vi "UI (Experienced).vi"() -> ()   [LabVIEW 2017, in "UI.lvlib"]
doc: "The Queued Message Handler of a Worker."
uses:
  UI.lvlib
  _support/Analysis Window Type.ctl
  _support/UI State.ctl
  1af51285-6659-428e-9c15-de70f1a207c9.vi
  1756710f-d813-4077-a3f9-6f06171a4225.vi
  b1498353-a107-4479-98d0-7e76c0451ff6.vi
  242d01f8-d211-4c25-bb6c-8191a2acbe42.vi
  da0d510b-1f54-4e49-9d1f-893e7e8abfcf.vi
  e403ca69-710b-4b23-8527-f02bfa86df9b.vi
  <userlib>/_NEVSTOP/Communicable State Machine(CSM)/AdvanceAPI/CSM - Revert Arguments-Safe String.vi
  <userlib>/_NEVSTOP/Communicable State Machine(CSM)/_Shared/Trim Single-line Text.vi
  <userlib>/_NEVSTOP/Communicable State Machine(CSM)/AdvanceAPI/CSM - Make String Arguments Safe.vi
  <userlib>/_NEVSTOP/Communicable State Machine(CSM)/AdvanceAPI/CSM - Break Down Multiple States String.vi
  <userlib>/_NEVSTOP/Communicable State Machine(CSM)/AdvanceAPI/CSM - Keywords.vi
  <userlib>/_NEVSTOP/Communicable State Machine(CSM)/addons/INI-Static-Variable-Support/_Support/instances/_CSM - Read File Logger Configuration - v1.0.vi
  <userlib>/_NEVSTOP/Communicable State Machine(CSM)/addons/API-String-Arugments-Support/_Support/Convert API String Arguments to Data(variant).vi
  <userlib>/_NEVSTOP/Communicable State Machine(CSM)/addons/API-String-Arugments-Support/_Support/Query Data as API String Arguments(variant).vi
  <userlib>/_NEVSTOP/Communicable State Machine(CSM)/addons/MassData-Parameter/_support/FGV-MassData(lvlibp).vi
  <userlib>/_NEVSTOP/Communicable State Machine(CSM)/_Polymophic/Add State(s) to Queue By BOOL(Element).vi
  <userlib>/_NEVSTOP/Communicable State Machine(CSM)/_Polymophic/CSM - Replace Marks in Messages.vi
  Acquisition/Acquisition.lvlib
  Logging/Logging.lvlib
  <userlib>/_NEVSTOP/Communicable State Machine(CSM)/Communicable State Machine.lvlib
  <userlib>/_NEVSTOP/Communicable State Machine(CSM)/addons/MassData-Parameter/CSM MassData Parameter Support.lvlib
  <userlib>/_NEVSTOP/Communicable State Machine(CSM)/addons/INI-Static-Variable-Support/INI-Static-Variable-Support.lvlib
  Algorithm/Algorithm.lvlib
  <userlib>/_NEVSTOP/Communicable State Machine(CSM)/addons/Logger/CSM File Logger.lvlib
  <userlib>/_NEVSTOP/Communicable State Machine(CSM)/addons/Watchdog/CSM Watchdog.lvlib
  <userlib>/_NEVSTOP/Communicable State Machine(CSM)/_Polymophic/Build Synchronous Message with Arguments.vi
panel:
  out "WaveformGraph":waveform(dbl)[](graph)
  in  "Analysis Window 1":T1
  out "AnalysisWnd 1":cluster{"f0":dbl, "df":dbl, "magnitude":dbl[]}[](graph)
  in  "Analysis Window 2":T1
  out "AnalysisWnd 2":cluster{"f0":dbl, "df":dbl, "magnitude":dbl[]}[](graph)
  in  "Settings":bool
  in  "Start":bool
  in  "Stop":bool
  out "Status":string
  in  "Exit":bool
  # "Continuous Measurement and Data Logger - CSM Version"
  # "Experienced Example"
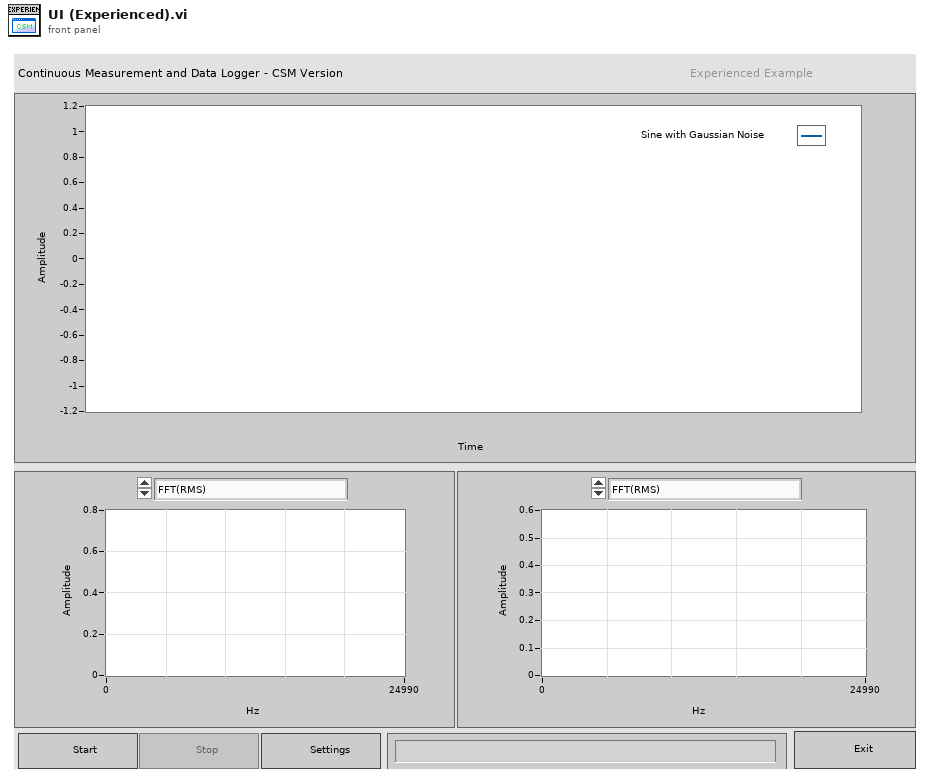
[diagram p1: front panel]
types:
  T1 = typedef "UI.lvlib/Analysis Window Type.ctl" = enum16{"FFT(RMS)", "FFT(Peak)", "Power Spectrum"}
  T2 = cluster{"Enable":bool, "Limit":cluster{"FileSize":i64, "FileNum":i32}, "Timestamp.Format":string, "AutoExit":bool}
  T3 = enum32{"Invalid", "Standard", "Closed", "Hidden", "Minimized", "Maximized"}
  T4 = enum32{"invalid app kind", "Development System", "Run Time System", "Student Edition", "Embedded LabVIEW", "Evaluation", "Custom"}
  T5 = typedef "UI.lvlib/UI State.ctl" = enum16{"Idle", "Acquiring and Logging", "Waiting for Exit", "Waiting for Exit (Acq Stopped)", "Waiting for Exit (Log Stopped)", "Waiting for Stop", "Waiting for Stop (Acq Stopped)", "Waiting for Stop (Log Stopped)"}
  T6 = enum32{"Invalid", "Default", "Floating", "Floating/Auto-Hide", "Modal"}
  T7 = typedef "Communicable State Machine.lvlib/_CSM_Response Source Message.ctl" = cluster{"‘State":string, "’Arguments":string, "’Error":errorcluster}
  T8 = cluster{"Current VI Reference":refnum<vi>, "Close Panel on Exit?":bool}
  T9 = cluster{"Core":cluster{"Current VI Reference":refnum<vi>, "Close Panel on Exit?":bool}, "UI Refs":cluster{"Start Ref":refnum<vi>, "Stop Ref":refnum<vi>, "Settings Ref":refnum<vi>, "Exit Ref":refnum<vi>, "Status Ref":refnum<vi>, "Data Ref":refnum<vi>, "Data Source Ref":refnum<vi>}, "State":T5, "Relationships":string}
  T10 = cluster{"Start Ref":refnum<vi>, "Stop Ref":refnum<vi>, "Settings Ref":refnum<vi>, "Exit Ref":refnum<vi>, "Status Ref":refnum<vi>, "Data Ref":refnum<vi>, "Data Source Ref":refnum<vi>}
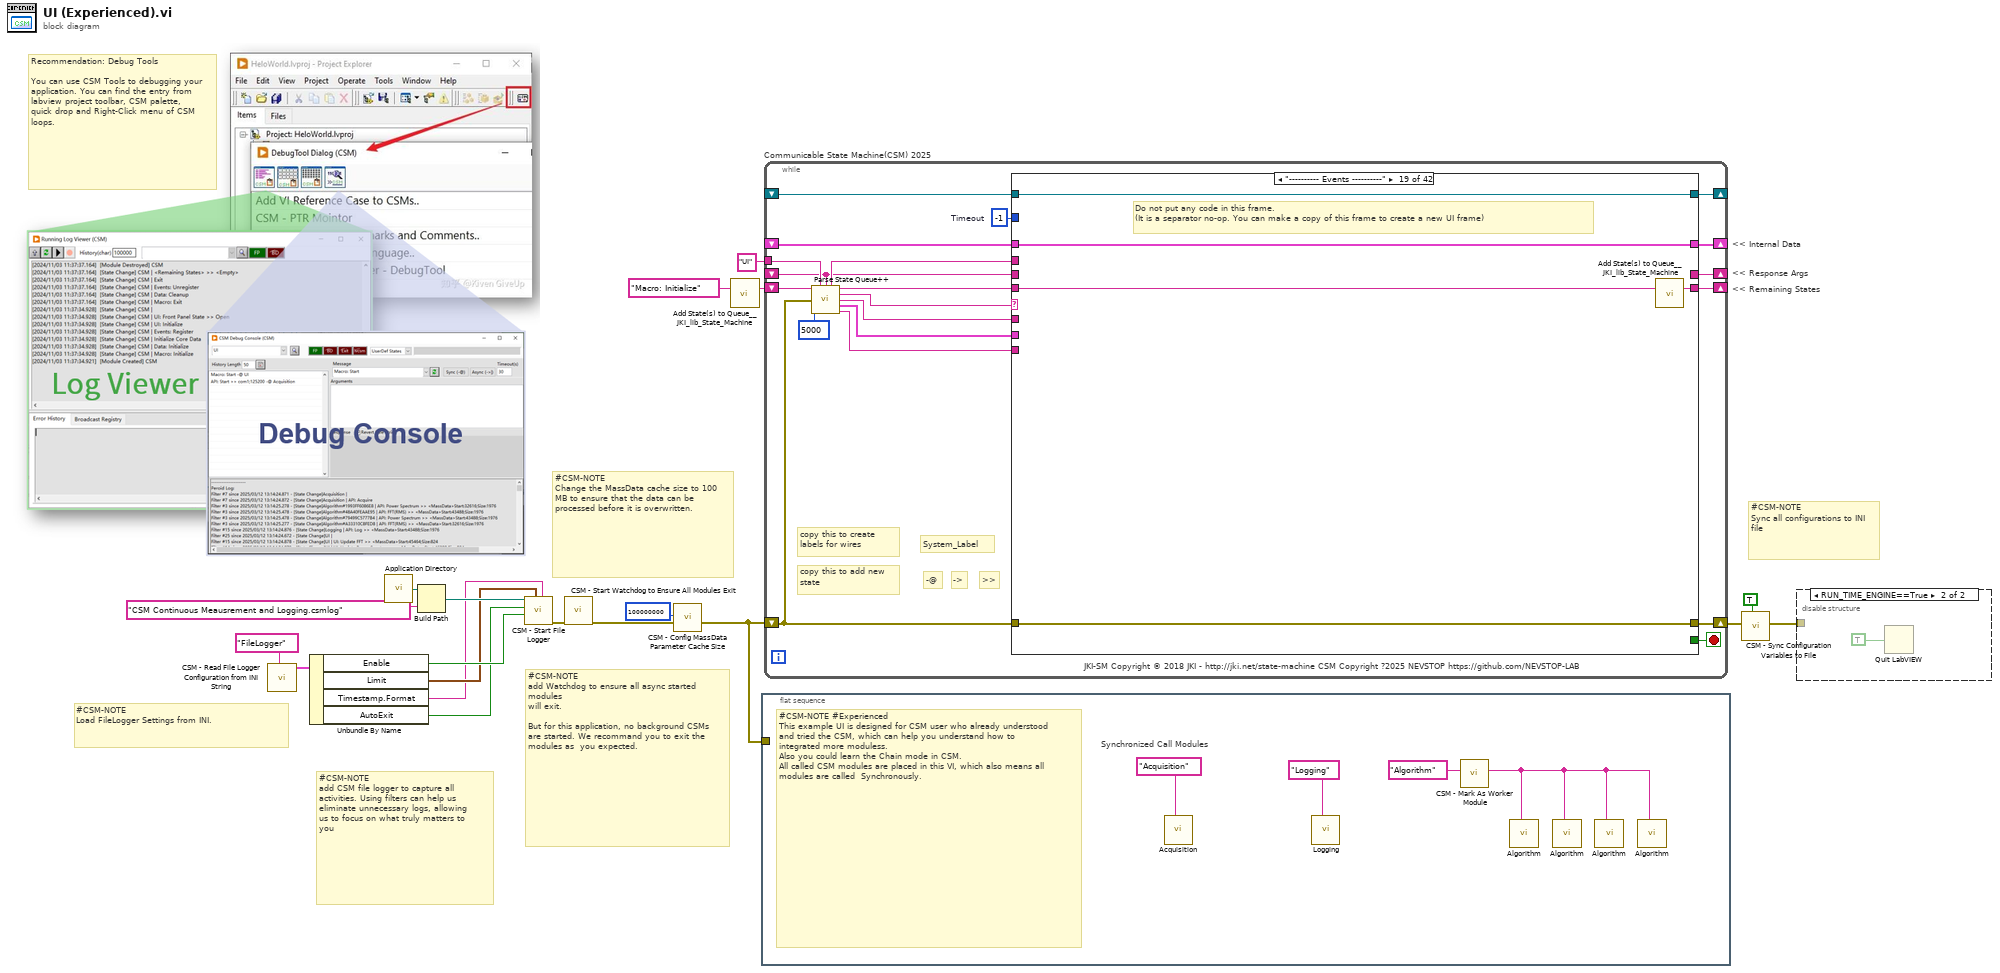
[diagram p0: block diagram]
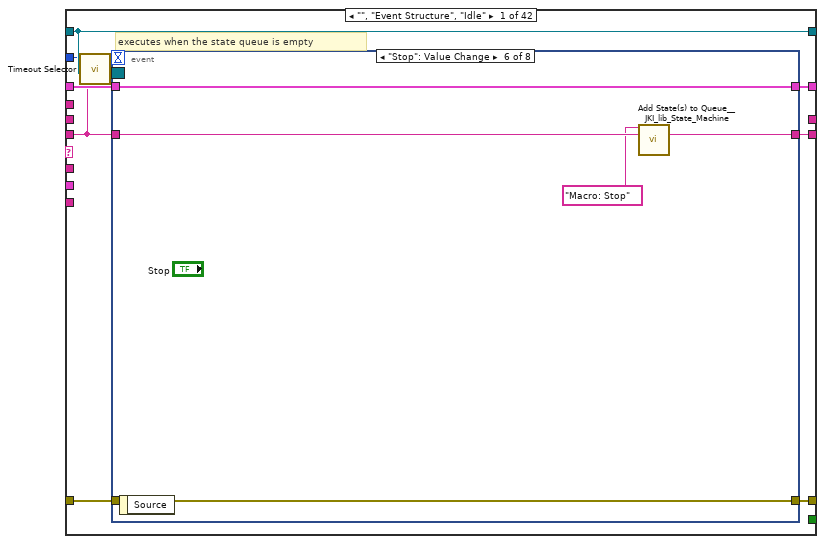
[diagram p3: hidden frame]
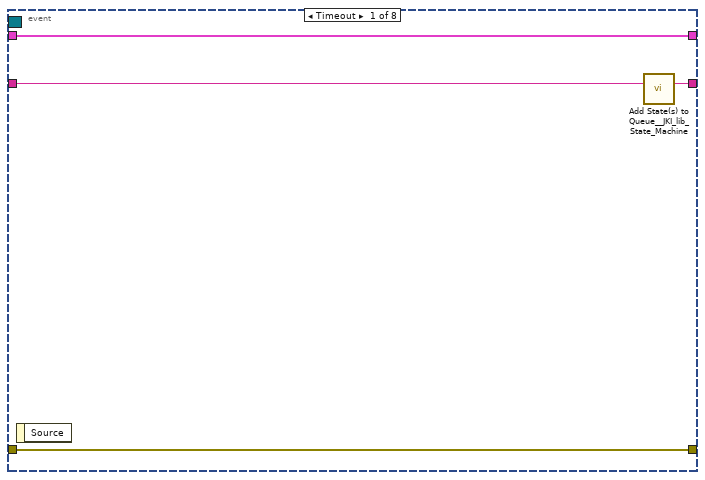
[diagram p4: hidden frame]
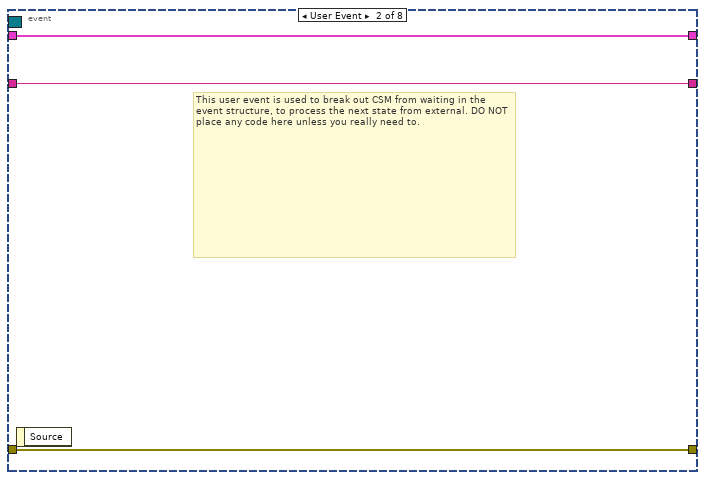
[diagram p5: hidden frame]
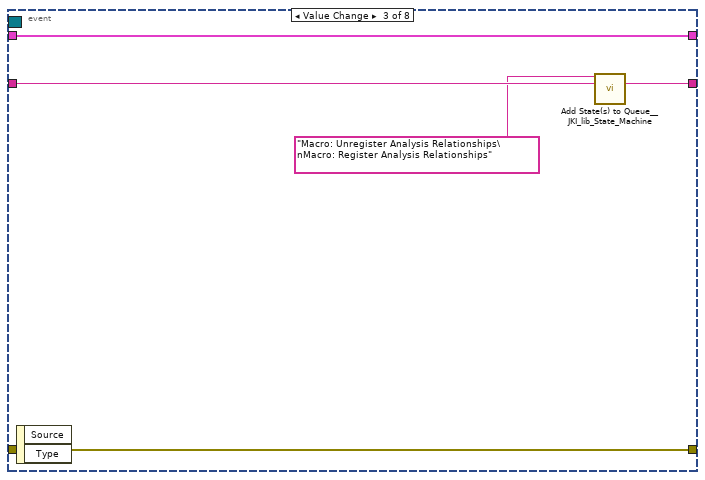
[diagram p6: hidden frame]
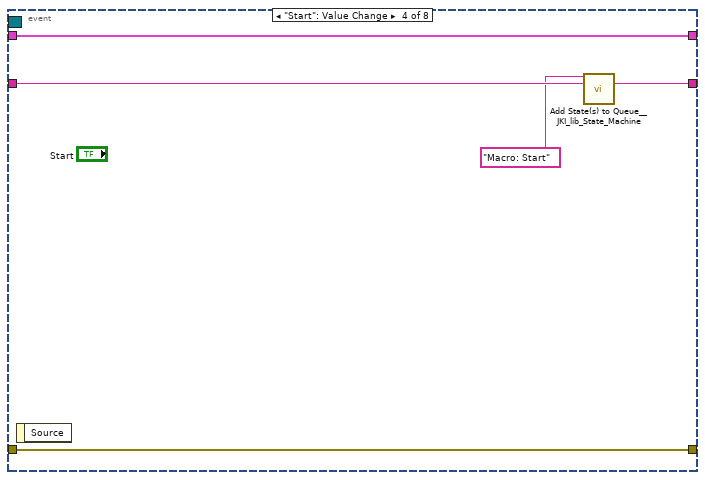
[diagram p7: hidden frame]
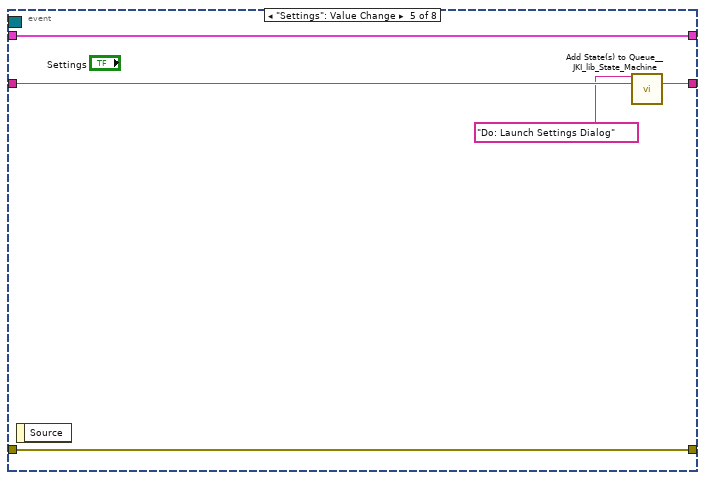
[diagram p8: hidden frame]
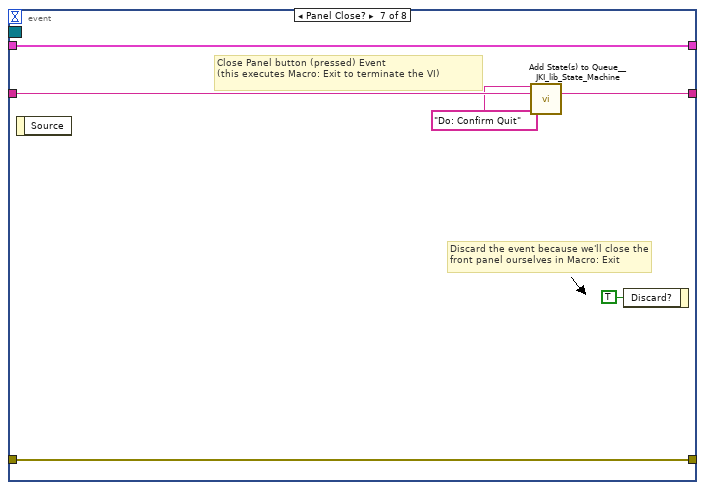
[diagram p9: hidden frame]
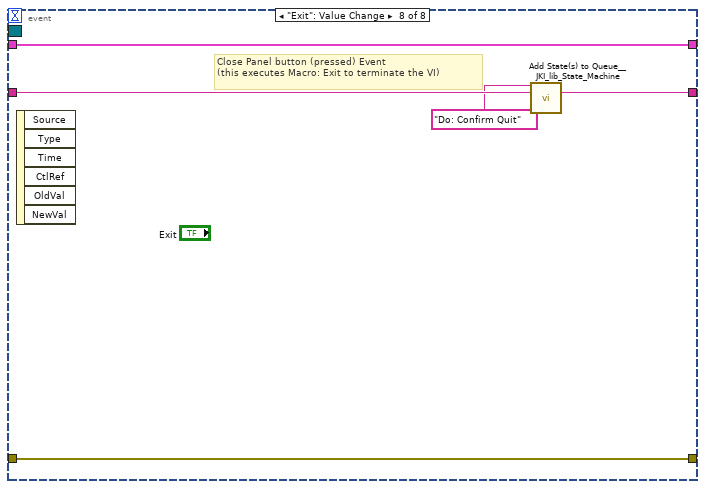
[diagram p10: hidden frame]
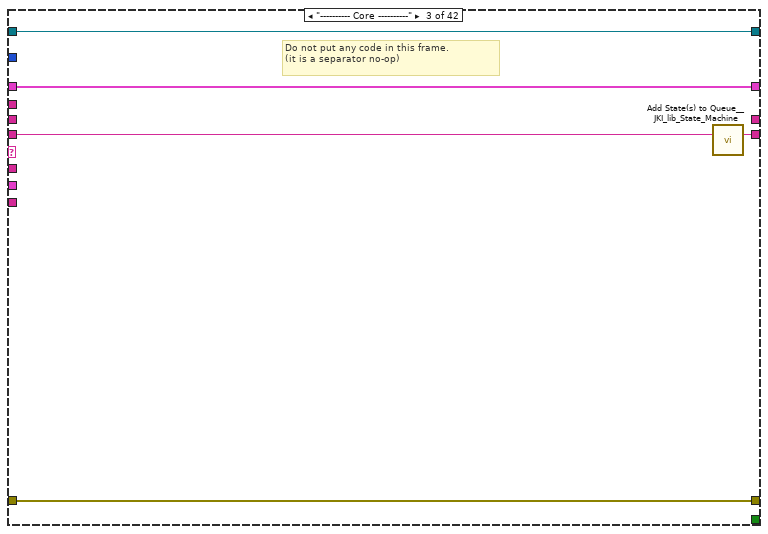
[diagram p12: hidden frame]
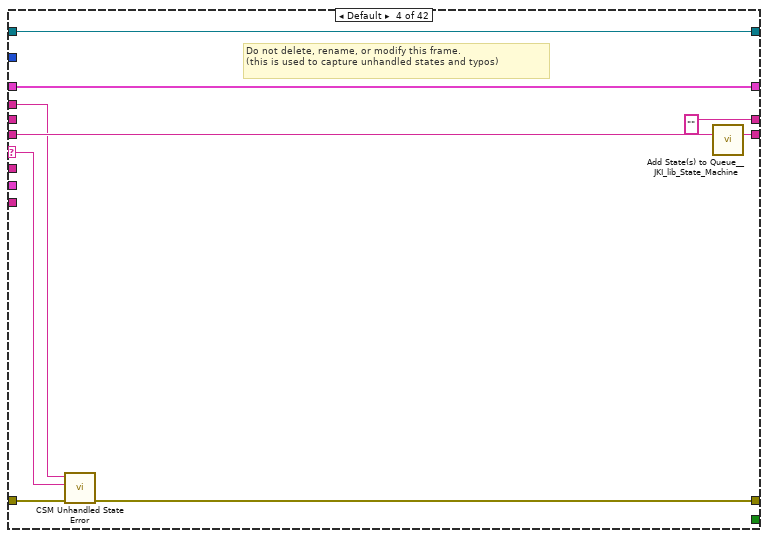
[diagram p13: hidden frame]
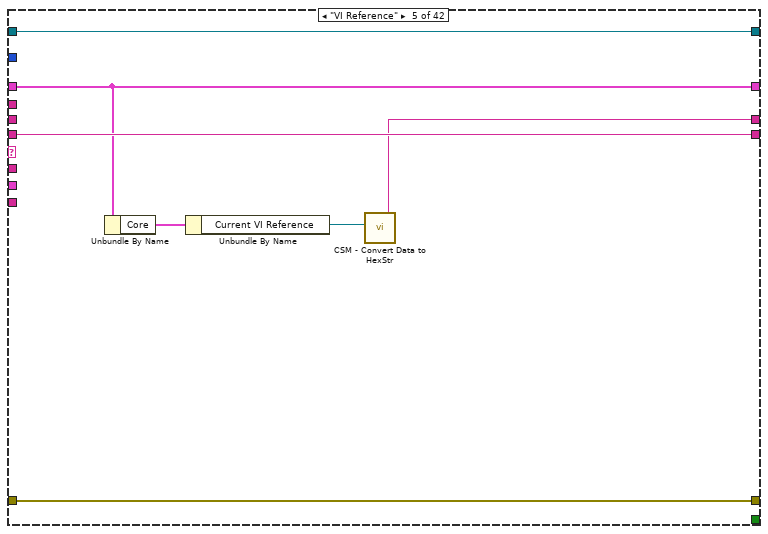
[diagram p14: hidden frame]
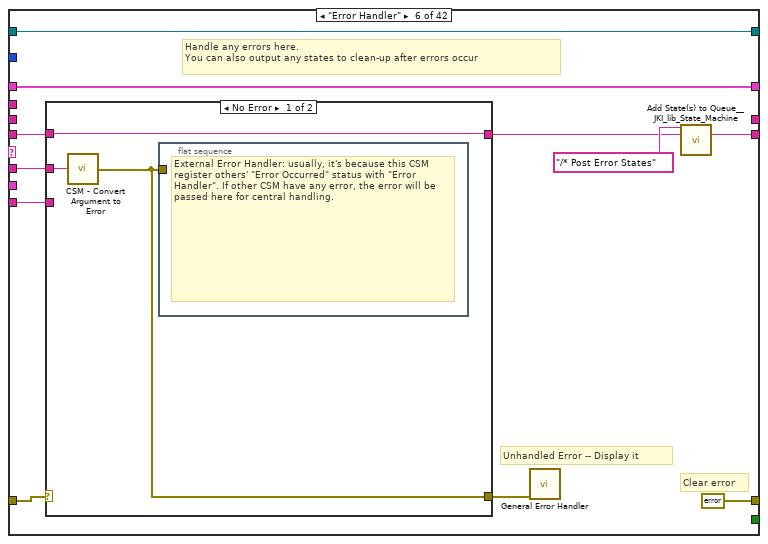
[diagram p15: hidden frame]
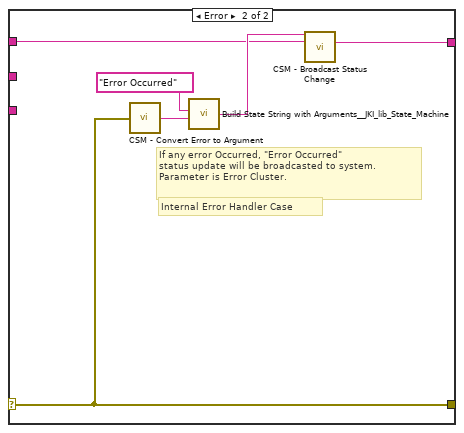
[diagram p16: hidden frame]
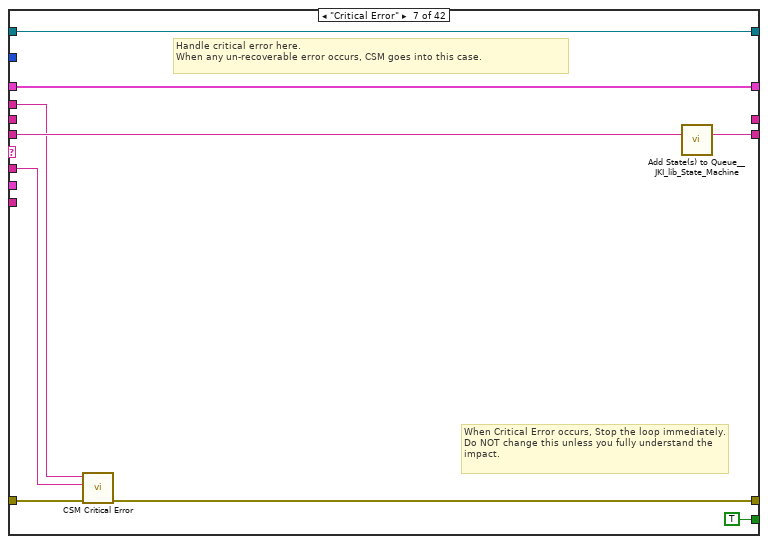
[diagram p17: hidden frame]
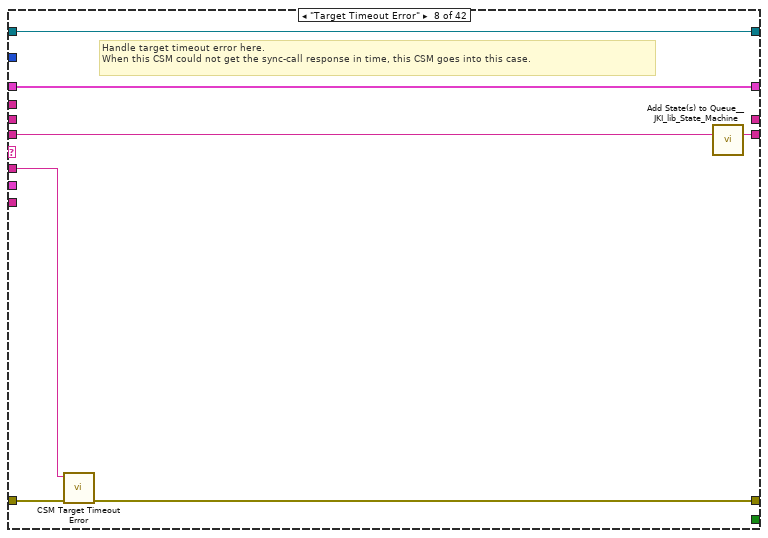
[diagram p18: hidden frame]
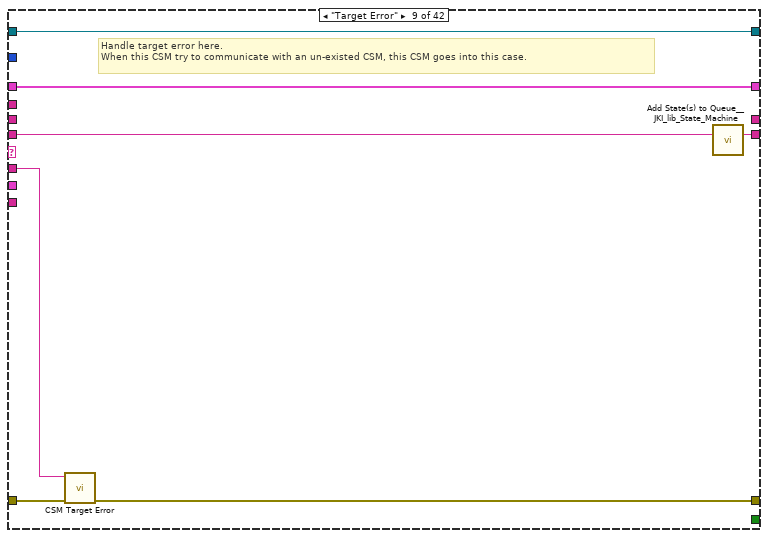
[diagram p19: hidden frame]
diagram:
  # "#CSM-NOTE\nSync all configurations to INI file"
  # "#CSM-NOTE\nChange the MassData cache size to 100 MB to ensure that the data can be processed before it is overwritten."
  # "Recommendation: Debug Tools\n\nYou can use CSM Tools to debugging your application. You can find the entry from labview project toolbar, CSM palette, quick drop and Right-Click menu of CSM loops."
  # "#CSM-NOTE\nLoad FileLogger Settings from INI."
  # "#CSM-NOTE\nadd CSM file logger to capture all activities. Using filters can help us eliminate unnecessary logs, allowing us to focus on what truly matters to you"
  # "#CSM-NOTE\nadd Watchdog to ensure all async started modules\nwill exit. \n\nBut for this application, no background CSMs are started. We recommand you to exit the modules as  you expected."
  # "<< Internal Data"
  # "<< Response Args"
  # "<< Remaining States"
  n1 = call-poly <userlib>:"CSM - Read File Logger Configuration from INI String.vi"("Section Name(\"FileLogger\")"="FileLogger" ("Section Name(\"\" as Default)")) -> ("FileLogger Configuration-v1"=w11:T2)  [unwired: 7 in, 1 out]
  n2 = Unbundle By Name(w11) -> ("Enable"=w10:bool, "Limit"=w9:cluster{"FileSize":i64, "FileNum":i32}, "Timestamp.Format"=w7:string, "AutoExit"=w8:bool)
  n3 = call <vilib>:"Application Directory.vi"() -> ("Application Directory"=w16:path)
  n4 = Build Path(base path=w16, name or relative path="CSM Continuous Meausrement and Logging.csmlog") -> (appended path=w14:path)
  n5 = call <userlib>:"CSM - Start File Logger.vi"("Timestamp Format"=w7, "Log Limit"=w9, "Watchdog? (T)"=w10, "Exit When All Module Exist? (F)"=w8, "Log File Path"=w14) -> ("error out"=w13:errorcluster)  [unwired: 4 in, 2 out]
  n6 = call <userlib>:"CSM - Start Watchdog to Ensure All Modules Exit.vi"("error in (no error)"=w13) -> ("error out"=w5:errorcluster)  [unwired: 10 in]
  n7 = call <userlib>:"CSM - Config MassData Parameter Cache Size.vi"("Error in"=w5, "Size (50M)"=100000000 ("size(1M)")) -> ("Error out"=w4:errorcluster)  [unwired: 9 in]
  n8 = call <vilib>:"Add State(s) to Queue__JKI_lib_State_Machine.vi"("State(s) in (\"\")"="Macro: Initialize") -> ("States Out"=w17:string)  [unwired: 14 in]
  n9 = flat-sequence {
    tunnel: w4 -> [_]
    frame #0 {
      # "#CSM-NOTE #Experienced\nThis example UI is designed for CSM user who already understood and tried the CSM, which can help you understand how to integrated more moduless.\nAlso you could learn the Chain mode in CSM.\nAll called CSM modules are placed in this VI, which also means all modules are called  Synchronously."
      # "Synchronized Call Modules"
      n10 = call "Acquisition.vi"("Name(\"\" to use uuid)"="Acquisition" ("Name(\"\" to use uuid)")) -> ()  [unwired: 11 in]
      n11 = call "Logging.vi"("Name(\"\" to use uuid)"="Logging" ("Name(\"\" to use uuid)")) -> ()  [unwired: 11 in]
      n12 = call <userlib>:"CSM - Mark As Worker Module.vi"("CSM Name"="Algorithm" ("Name(\"\" to use uuid)")) -> ("CSM Name (Marked As Worker)"=w21:string)  [unwired: 9 in]
      n13 = call "Algorithm.vi"("Name(\"\" to use uuid)"=w21) -> ()  [unwired: 11 in]
      n14 = call "Algorithm.vi"("Name(\"\" to use uuid)"=w21) -> ()  [unwired: 11 in]
      n15 = call "Algorithm.vi"("Name(\"\" to use uuid)"=w21) -> ()  [unwired: 11 in]
      n16 = call "Algorithm.vi"("Name(\"\" to use uuid)"=w21) -> ()  [unwired: 11 in]
    }
  }
  n17 = while "Communicable State Machine(CSM) 2025" {
    shift-right: [w39] -> _
    shift-left: _ -> [w38]
    shift-right: [w41] -> w2
    shift-left: w4 -> [w36]
    shift-right: [w40] -> _
    shift-left: w17 -> [w42]
    tunnel: "UI" ("Name(\"\" to use uuid)") -> [w31]
    shift-right: [w34] -> _
    shift-left: _ -> [w26]
    shift-right: [w33] -> _
    shift-left: _ -> [w32]
    stop <- w24 stop-if-true
    w37 = -1  # Timeout
    # "JKI-SM Copyright © 2018 JKI - http://jki.net/state-machine CSM Copyright ?2025 NEVSTOP https://github.com/NEVSTOP-LAB"
    # "copy this to add new state"
    # ">>"
    # "->"
    # "-@"
    # "copy this to create labels for wires"
    # "System_Label"
    n18 = call <userlib>:"Parse State Queue++.vi"("State Queue"=w42, "Name (\"\" to Use UUID)"=w31, "Response Arguments"=w26, "Previous Error"=w36, "Response Timeout (-2 Use Global Settings)"=5000 ("Response Timeout(1000ms)")) -> ("Name Used"=w27:string, "Remaining States"=w43:string, "Current State"=w30:string, "Arguments"=w25:string, "Additional Information"=w29:T7, "Source CSM"=w28:string)  [unwired: 5 in]
    n19 = case shown="\"---------- Events ----------\"" w30 {
      selector: w30 -> [_ _ _ w101 _ _ _ _ _ _ _ _ _ _ _ _ _ _ _ _ _ _ _ _ _ _ _ _ _ _ _ _ _ _ _ _ _ _ _ _ _ _]
      tunnel: w43 -> [w44 w93 w99 w107 w114 w119 w142 w150 w157 w161 w165 w180 w187 w192 w201 w207 w214 w221 w226 w232 w236 w242 w262 w276 w289 w297 w313 w387 w396 w409 w416 w421 w428 w436 w444 w455 w466 w484 w509 w515 w523 w561]
      tunnel: w25 -> [_ _ _ _ _ w117 w136 w146 w153 _ _ _ _ _ _ w205 w211 _ _ _ _ _ _ _ _ w292 w307 w382 w400 w406 w413 _ _ _ _ _ _ _ _ w510 _ _]
      tunnel: w38 -> [w51 w92 w96 w105 w113 w125 w143 w148 w155 w160 w164 w173 w185 w189 _ w204 w212 w216 w223 w231 w235 w239 w248 w266 w279 w295 w309 w385 w402 w408 w415 w418 w425 w439 w451 w458 w462 w482 w506 w512 w516 w556]
      tunnel: [w50 w94 w97 w100 w115 errorcluster {"status"=FALSE, "code"=0, "source"=""} ("error out") w138 w145 w152 w162 w166 w177 w184 w190 w195 w203 w210 w217 w224 w227 w234 w240 w260 w277 w290 w293 w310 w379 w398 w405 w412 w419 w426 w440 w453 w461 w470 _ w507 w513 w517 _] -> w41
      tunnel: w36 -> [w49 w94 w97 w108 w115 w123 w144 w151 w158 w162 w166 w177 w184 w190 w195 _ _ w218 w224 _ w237 w240 w260 w277 w290 w294 w311 _ _ _ _ w419 w426 w440 w453 w461 w470 _ w507 w513 _ _]
      tunnel: [w52 w93 w98 w106 w114 w121 w141 w149 w156 w161 w165 w179 w186 w191 w200 w207 w214 w220 w225 w232 w236 w241 w261 w276 w289 w296 w312 w387 w397 w409 w416 w420 w427 w437 w445 w456 w467 w483 w508 w514 w523 w554] -> w40
      tunnel: [_ _ _ _ _ _ TRUE _ _ _ _ _ TRUE _ _ _ _ _ _ _ _ _ _ _ _ _ _ _ _ _ _ _ _ _ _ _ _ _ _ _ _ _] -> w24
      tunnel: [w48 w92 w96 w105 w113 w125 w143 w148 w155 w160 w164 w178 w185 w189 w194 w202 w208 w216 w223 w231 w235 w239 w247 w266 w279 w295 w309 w385 w402 w408 w415 w418 w425 w435 w442 w457 w468 w482 w506 w512 w516 w555] -> w39
      tunnel: w37 -> [w46 _ _ _ _ _ _ _ _ _ _ _ _ _ _ _ _ _ _ _ _ _ _ _ _ _ _ _ _ _ _ _ _ _ _ _ _ _ _ _ _ _]
      tunnel: w28 -> [_ _ _ _ _ w116 _ _ _ _ _ _ _ _ _ _ _ _ _ _ _ _ _ _ _ _ _ _ _ _ _ _ _ _ _ _ _ _ _ _ _ _]
      tunnel: w29 -> [_ _ _ _ _ _ _ _ _ _ _ _ _ _ _ _ _ _ _ _ _ _ _ _ _ _ _ _ _ _ _ _ _ _ _ _ _ _ _ _ _ _]
      tunnel: [_ _ _ "" w109 _ _ _ _ _ _ _ _ _ _ _ w209 _ _ _ _ _ _ _ _ _ _ _ _ _ _ _ _ _ _ _ _ _ _ _ _ _] -> w34
      tunnel: [w47 w91 w95 w103 w112 w124 w139 w147 w154 w159 w163 w167 w182 w188 w198 w206 w213 w215 w222 w230 w233 w238 w259 w275 w288 w291 w306 w386 w401 w407 w414 w417 w424 w438 w452 w460 w469 w475 w505 w511 w524 w560] -> w33
      tunnel: w32 -> [w47 w91 w95 w103 w112 w124 w139 w147 w154 w159 w163 w167 w182 w188 w198 w206 w213 w215 w222 _ w233 w238 w259 w275 w288 w291 w306 w386 w401 w407 w414 w417 w424 w438 w452 w460 w469 w475 w505 w511 w524 w560]
      tunnel: w27 -> [_ _ _ w102 _ _ w137 _ _ _ _ _ _ _ _ _ _ _ _ w229 _ _ _ _ _ _ _ _ _ _ _ _ _ _ _ _ _ w473 _ _ w519 _]
      tunnel: w26 -> [_ _ _ _ _ _ _ _ _ _ _ _ _ _ _ _ _ _ _ _ _ _ _ _ _ _ _ _ _ _ _ _ _ _ _ _ _ _ _ _ _ _]
      frame "", "Event Structure", "Idle" {
        # "executes when the state queue is empty"
        n20 = call <userlib>:"Timeout Selector.vi"("Remaining States"=w44, "Timeout Expected"=w46) -> ("Timeout"=w45:i32)  [unwired: 5 in]
        n21 = event shown="[5] \"Stop\": Value Change" {
          selector: w47 -> [_ _ _ _ _ _ _ _]
          dyn-events: _ -> [_ _ _ _ _ _ _ _]
          timeout: w45 -> [_ _ _ _ _ _ _ _]
          tunnel: w44 -> [w56 w58 w61 w66 w71 w76 w85 w90]
          tunnel: [w55 w58 w62 w67 w72 w77 w84 w89] -> w52
          tunnel: w51 -> [w53 w59 w63 w68 w73 w78 w82 w87]
          tunnel: [w54 w57 w64 w69 w74 w79 w83 w88] -> w50
          tunnel: w49 -> [w54 w57 w64 w69 w74 w79 w83 w88]
          tunnel: [w53 w59 w63 w68 w73 w78 w82 w87] -> w48
          event Timeout {
            n22 = event-data() -> ()  [unwired: 1 in, 1 out]
            n23 = call <vilib>:"Add State(s) to Queue__JKI_lib_State_Machine.vi"("State(s) in (\"\")"=w56) -> ("States Out"=w55:string)  [unwired: 14 in]
          }
          event User Event {
            # "This user event is used to break out CSM from waiting in the event structure, to process the next state from external. DO NOT place any code here unless you really need to."
            n24 = event-data() -> ()  [unwired: 1 in, 1 out]
          }
          event Value Change {
            n25 = event-data() -> ()  [unwired: 1 in, 2 out]
            n26 = call <vilib>:"Add State(s) to Queue__JKI_lib_State_Machine.vi"("State(s) in Front (\"\")"="Macro: Unregister Analysis Relationships\nMacro: Register Analysis Relationships" ("State(s) in Front (\"\")"), "State(s) in (\"\")"=w61) -> ("States Out"=w62:string)  [unwired: 13 in]
          }
          event "Start": Value Change {
            n27 = event-data() -> ()  [unwired: 1 in, 1 out]
            n28 = call <vilib>:"Add State(s) to Queue__JKI_lib_State_Machine.vi"("State(s) in Front (\"\")"="Macro: Start" ("State(s) in Front (\"\")"), "State(s) in (\"\")"=w66) -> ("States Out"=w67:string)  [unwired: 13 in]
          }
          event "Settings": Value Change {
            n29 = event-data() -> ()  [unwired: 1 in, 1 out]
            n30 = call <vilib>:"Add State(s) to Queue__JKI_lib_State_Machine.vi"("State(s) in Front (\"\")"="Do: Launch Settings Dialog" ("State(s) in Front (\"\")"), "State(s) in (\"\")"=w71) -> ("States Out"=w72:string)  [unwired: 13 in]
          }
          event "Stop": Value Change {
            n31 = event-data() -> ()  [unwired: 1 in, 1 out]
            n32 = call <vilib>:"Add State(s) to Queue__JKI_lib_State_Machine.vi"("State(s) in Front (\"\")"="Macro: Stop" ("State(s) in Front (\"\")"), "State(s) in (\"\")"=w76) -> ("States Out"=w77:string)  [unwired: 13 in]
          }
          event Panel Close? {
            # "Discard the event because we'll close the front panel ourselves in Macro: Exit"
            # "Close Panel button (pressed) Event\n(this executes Macro: Exit to terminate the VI)"
            n33 = event-data() -> ()  [unwired: 1 in, 1 out]
            n34 = call <vilib>:"Add State(s) to Queue__JKI_lib_State_Machine.vi"("State(s) in Front (\"\")"="Do: Confirm Quit", "State(s) in (\"\")"=w85) -> ("States Out"=w84:string)  [unwired: 13 in]
            n35 = event-data("Discard?"=TRUE) -> ()  [unwired: 1 in, 1 out]
          }
          event "Exit": Value Change {
            # "Close Panel button (pressed) Event\n(this executes Macro: Exit to terminate the VI)"
            n36 = event-data() -> ()  [unwired: 1 in, 6 out]
            n37 = call <vilib>:"Add State(s) to Queue__JKI_lib_State_Machine.vi"("State(s) in Front (\"\")"="Do: Confirm Quit", "State(s) in (\"\")"=w90) -> ("States Out"=w89:string)  [unwired: 13 in]
          }
        }
      }
      frame "CSM Documentation" {
        # "CSM Documentation"
        # "State Syntax:\nStateCategory: State >> Argument -@ CSMName\nStateCategory: State >> Argument -> CSMName\n\nLine Terminator: Line feed"
        # "Commenting:\nTo add a comment use \"//\" or \"#\" and all text to the right will be ignored\nCommenting Example:\nUI: Initialize // This initializes the UI\n// Another comment line"
        # "Example:\nUI: Help >> About -@Main\nUI: Help >> About ->Main\n\nWhere \"UI\" is the state category\nWhere \"Help\" is the state\nWhere \"About\" is the argument\nWhere \"Main\" is the Name of CSM,which actually run the \"UI: Help >> About\"\n\n    \"-@\" stands for sync state. Current CSM will wait until the state is finished. \n            - if \"Main\" named CSM does not exist, \"Target Error\" will occur.\n            - if \"Main\" named CSM is in another sync remote state, \"Target Busy Error\" will occur.\n            - if \"Main\" named CSM could not finish the state in time, \"Target Timeout Error\" will occur.\n            - if everything is right. \"Response\" will occur with Argument back from \"Main\" named CSM. \n\n    \"->\" stands for async state. Current CSM will post the state and continue to next state in next iteration.\n            - if \"Main\" named CSM does not exist, \"Target Error\" will occur.\n            - if everything is right. \"Async Message Posted\" will occur.\n            - After State is finished. Caller will receive a \"Async Response\" state from callee.\n\nWhen duplicated name is used for multiple CSM module or some framework problem happens, \"Critical Error\" will occur."
      }
      frame "---------- Core ----------" {
        # "Do not put any code in this frame.\n(it is a separator no-op)"
        n38 = call <vilib>:"Add State(s) to Queue__JKI_lib_State_Machine.vi"("State(s) in (\"\")"=w99) -> ("States Out"=w98:string)  [unwired: 14 in]
      }
      frame Default {
        # "Do not delete, rename, or modify this frame.\n(this is used to capture unhandled states and typos)"
        n39 = call <userlib>:"CSM Unhandled State Error.vi"("error in (no error)"=w108, "Undefined State"=w101, "CSM Name"=w102) -> ("error out"=w100:errorcluster)  [unwired: 8 in]
        n40 = call <vilib>:"Add State(s) to Queue__JKI_lib_State_Machine.vi"("State(s) in (\"\")"=w107) -> ("States Out"=w106:string)  [unwired: 14 in]
      }
      frame "VI Reference" {
        n41 = Unbundle By Name(w113) -> ("Core"=w111:T8)
        n42 = Unbundle By Name(w111) -> ("Current VI Reference"=w110:refnum<vi>)
        n43 = call <userlib>:"CSM - Convert Data to HexStr.vi"("Variant"=w110) -> ("HEX String (0-9,A-F)"=w109:string)  [unwired: 8 in]
      }
      frame "Error Handler" {
        # "Unhandled Error -- Display it"
        # "Handle any errors here.\nYou can also output any states to clean-up after errors occur"
        # "Clear error"
        n44 = case shown="No Error" w123 {
          selector: w123 -> [_ w130]
          tunnel: [w128 w132] -> w120
          tunnel: w119 -> [w128 w131]
          tunnel: [w127 w130] -> w118
          tunnel: w117 -> [w129 _]
          tunnel: w116 -> [_ _]
          frame No Error {
            n45 = call <userlib>:"CSM - Convert Argument to Error.vi"("Argument"=w129) -> ("Error"=w127:errorcluster)  [unwired: 4 in]
            n46 = flat-sequence {
              tunnel: w127 -> [_]
              frame #0 {
                # "External Error Handler: usually, it's because this CSM register others' \"Error Occurred\" status with \"Error Handler\". If other CSM have any error, the error will be passed here for central handling."
              }
            }
          }
          frame Error {
            # "Internal Error Handler Case"
            # "If any error Occurred, \"Error Occurred\" \nstatus update will be broadcasted to system.\nParameter is Error Cluster."
            n47 = call <userlib>:"CSM - Convert Error to Argument.vi"("Error"=w130) -> ("Argument"=w134:string)  [unwired: 4 in]
            n48 = call <vilib>:"Build State String with Arguments__JKI_lib_State_Machine.vi"("Arguments (\"\")"=w134, "State"="Error Occurred" ("Status with Arguments")) -> ("State with Arguments"=w133:string)  [unwired: 4 in]
            n49 = call <userlib>:"CSM - Broadcast Status Change.vi"("Status With Arguments"=w133, "State Queue"=w131) -> ("Remaining States"=w132:string)  [unwired: 13 in]
          }
        }
        n50 = call <vilib>:"General Error Handler.vi"("error in (no error)"=w118) -> ()  [unwired: 10 in, 5 out]
        n51 = call <vilib>:"Add State(s) to Queue__JKI_lib_State_Machine.vi"("State(s) in Front (\"\")"="/* Post Error States", "State(s) in (\"\")"=w120) -> ("States Out"=w121:string)  [unwired: 13 in]
      }
      frame "Critical Error" {
        # "Handle critical error here.\nWhen any un-recoverable error occurs, CSM goes into this case."
        # "When Critical Error occurs, Stop the loop immediately. Do NOT change this unless you fully understand the impact."
        n52 = call <userlib>:"CSM Critical Error.vi"("error in (no error)"=w144, "Arugments (As Reason)"=w136, "CSM Name"=w137) -> ("error out"=w138:errorcluster)  [unwired: 8 in]
        n53 = call <vilib>:"Add State(s) to Queue__JKI_lib_State_Machine.vi"("State(s) in (\"\")"=w142) -> ("States Out"=w141:string)  [unwired: 14 in]
      }
      frame "Target Timeout Error" {
        # "Handle target timeout error here.\nWhen this CSM could not get the sync-call response in time, this CSM goes into this case."
        n54 = call <userlib>:"CSM Target Timeout Error.vi"("error in (no error)"=w151, "Arguments (As CSM Name)"=w146) -> ("error out"=w145:errorcluster)  [unwired: 9 in]
        n55 = call <vilib>:"Add State(s) to Queue__JKI_lib_State_Machine.vi"("State(s) in (\"\")"=w150) -> ("States Out"=w149:string)  [unwired: 14 in]
      }
      frame "Target Error" {
        # "Handle target error here.\nWhen this CSM try to communicate with an un-existed CSM, this CSM goes into this case."
        n56 = call <userlib>:"CSM Target Error.vi"("error in (no error)"=w158, "Arguments (As CSM Name)"=w153) -> ("error out"=w152:errorcluster)  [unwired: 9 in]
        n57 = call <vilib>:"Add State(s) to Queue__JKI_lib_State_Machine.vi"("State(s) in (\"\")"=w157) -> ("States Out"=w156:string)  [unwired: 14 in]
      }
      frame "Async Response", "Response" {
        # "Handle Async-call Response (\"Async Response\" for ->)"
        # "Handle Sync-call Response (\"Response\" for -@)"
        # "After Message is executed, CSM+ goes to this state for receive the response. \n    For Async Message(->), \"Async Response\" is used. This CSM will goes to \"Async Message Posted\" immediately and receive the \"Async Response\" after the callee finishes the message.\n    For Sync Message(@),  This CSM will wait until the message is done and immediately goes to \"Response\""
      }
      frame "Async Message Posted" {
        # "Handle post action for async message (->)."
        # "After Async Message is posted (->), CSM+ goes to this state for post-action. You can use Argument - State to tell which Async Message is called."
      }
      frame "Initialize Core Data" {
        # "Do not delete, rename, or modify this frame.\n(this is used to determine panel behavior on exit)"
        # "originally closed?"
        # "exe?"
        # "If panel starts closed or is an EXE, then close it when we exit"
        n58 = property class="VI"() -> ("FP.State"=w170:T3)  [unwired: 2 in, 2 out]
        n59 = property class="App"() -> ("App.Kind"=w176:T4)  [unwired: 2 in, 2 out]
        n60 = control-ref of="Current VI Reference"() -> (w171:refnum<vi>)
        n61 = Equal?(x=w170, y=T3."Closed" ("Front Panel Window:State")) -> (x = y?=w168:bool)
        n62 = Equal?(x=w176, y=T4."Run Time System" ("Application:Kind")) -> (x = y?=w174:bool)
        n63 = Or(x=w168, y=w174) -> (x .or. y?=w172:bool)
        n64 = Bundle By Name(cluster=w173, "Core.Current VI Reference"=w171, "Core.Close Panel on Exit?"=w172) -> (w178:T9)
        n65 = call <vilib>:"Add State(s) to Queue__JKI_lib_State_Machine.vi"("State(s) in (\"\")"=w180) -> ("States Out"=w179:string)  [unwired: 14 in]
      }
      frame "Exit" {
        # "Do not put any code in this frame.\n(No errors that occur here will be handled.)"
        n66 = local write "Status"("Exit" ("Exit String")) -> ()
        n67 = call <vilib>:"Add State(s) to Queue__JKI_lib_State_Machine.vi"("State(s) in (\"\")"=w187) -> ("States Out"=w186:string)  [unwired: 14 in]
      }
      frame "---------- Data ----------" {
        # "Do not put any code in this frame.\n(It is a separator no-op. You can make a copy of this frame to create a new Data frame)"
        n68 = call <vilib>:"Add State(s) to Queue__JKI_lib_State_Machine.vi"("State(s) in (\"\")"=w192) -> ("States Out"=w191:string)  [unwired: 14 in]
      }
      frame "Data: Initialize" {
        w193 = ""  # Relationships
        w196 = UI_State."Idle"  # State
        w197 = T10 {"Start Ref"=refnum, "Stop Ref"=refnum, "Settings Ref"=refnum, "Exit Ref"=refnum, "Status Ref"=refnum, "Data Ref"=refnum, "Data Source Ref"=refnum}  # UI Refs
        w199 = T8 {"Current VI Reference"=refnum, "Close Panel on Exit?"=FALSE}  # Core
        # "Initialize the shift-register data, here.\n(data names are defined by what you wire into the bundle function)"
        n69 = Bundle("Core"=w199, "UI Refs"=w197, "State"=w196, "Relationships"=w193) -> (w194:T9)  [unwired: 1 in]
        n70 = call <vilib>:"Add State(s) to Queue__JKI_lib_State_Machine.vi"("State(s) in (\"\")"=w201) -> ("States Out"=w200:string)  [unwired: 14 in]
      }
      frame "Data: Set Configuration" {
        n71 = call "Convert API String Arguments to Data.vim"("Reference Type"=w204, "API String"=w205) -> ("error out"=w203:errorcluster, "Data"=w202:T9)  [unwired: 6 in]
      }
      frame "Data: Get Configuration", "Data: Get Internal Data" {
        n72 = call "Query Data as API String Arguments.vim"("Name"=w211, "Cluster Data"=w212) -> ("error"=w210:errorcluster, "API String"=w209:string, "Cluster Data (dup)"=w208:T9)  [unwired: 7 in]
      }
      frame "Data: Cleanup" {
        # "Cleanup any data and references, here.\n(this is called automatically, by the Macro: Exit)"
        n73 = Unbundle By Name(w216) -> ("Core.Current VI Reference"=w219:refnum<vi>)
        n74 = Close Reference(reference=w219, error in (no error)=w218) -> (error out=w217:errorcluster)
        n75 = call <vilib>:"Add State(s) to Queue__JKI_lib_State_Machine.vi"("State(s) in (\"\")"=w221) -> ("States Out"=w220:string)  [unwired: 14 in]
      }
      frame "---------- Events ----------" {
        # "Do not put any code in this frame.\n(It is a separator no-op. You can make a copy of this frame to create a new UI frame)"
        n76 = call <vilib>:"Add State(s) to Queue__JKI_lib_State_Machine.vi"("State(s) in (\"\")"=w226) -> ("States Out"=w225:string)  [unwired: 14 in]
      }
      frame "Events: Register" {
        # "Register message event to break Waiting in Event structure."
        n77 = call <userlib>:"CSM - Get New State Notifier Event.vi"("Name (\"\" to Use UUID)"=w229) -> ("error out"=w227:errorcluster, "New State Notifier Event"=w228:refnum<user-event>)  [unwired: 9 in]
        n78 = register-events(w228) -> (reference out=w230:refnum<event-registration>)  [unwired: 2 in, 1 out]
      }
      frame "Events: Unregister" {
        n79 = Unregister For Events(event registration refnum=w233, error in=w237) -> (error out=w234:errorcluster)
      }
      frame "---------- UI ----------" {
        # "Do not put any code in this frame.\n(It is a separator no-op. You can make a copy of this frame to create a new UI frame)"
        n80 = call <vilib>:"Add State(s) to Queue__JKI_lib_State_Machine.vi"("State(s) in (\"\")"=w242) -> ("States Out"=w241:string)  [unwired: 14 in]
      }
      frame "UI: Initialize" {
        w243 = cluster{"f0":dbl, "df":dbl, "magnitude":dbl[]}[] [] ("FFT")
        # "Initialize the User Interface, here.\n(this is called automatically, by the Macro: Init)"
        n81 = control-ref of="WaveformGraph"() -> (w251:refnum<vi>)
        n82 = property on="AnalysisWnd 1" class="WFGraph (strict)"("Value"=w243) -> ()  [unwired: 2 in, 2 out]
        n83 = property on="AnalysisWnd 2" class="WFGraph (strict)"("Value"=w243) -> ()  [unwired: 2 in, 2 out]
        n84 = property on="WaveformGraph" class="WFChart (strict)"("History Data"=waveform(dbl)[][] []) -> ()  [unwired: 2 in, 2 out]
        n85 = control-ref of="Start"() -> (w256:refnum<vi>)
        n86 = control-ref of="Stop"() -> (w255:refnum<vi>)
        n87 = control-ref of="Settings"() -> (w257:refnum<vi>)
        n88 = control-ref of="Exit"() -> (w258:refnum<vi>)
        n89 = control-ref of="Status"() -> (w252:refnum<vi>)
        n90 = Bundle By Name(cluster=w248, "UI Refs.Start Ref"=w256, "UI Refs.Stop Ref"=w255, "UI Refs.Settings Ref"=w257, "UI Refs.Exit Ref"=w258, "UI Refs.Status Ref"=w252, "UI Refs.Data Ref"=w251) -> (w247:T9)
        n91 = Build Array(w256, w258, w257) -> (w254:refnum<vi>[])
        n92 = Build Array(w255) -> (w253:refnum<vi>[])
        n93 = local write "Analysis Window 1"(Analysis_Window_Type."FFT(RMS)" ("Analysis Window 1")) -> ()
        n94 = local write "Analysis Window 2"(Analysis_Window_Type."Power Spectrum" ("Analysis Window 2")) -> ()
        n95 = call "Set Enable State on Multiple Controls.vi"("Enable?"=TRUE, "Controls"=w254) -> ()  [unwired: 10 in]
        n96 = call "Set Enable State on Multiple Controls.vi"("Enable?"=FALSE, "Controls"=w253) -> ()  [unwired: 10 in]
        n97 = call <vilib>:"Add State(s) to Queue__JKI_lib_State_Machine.vi"("State(s) in (\"\")"=w262) -> ("States Out"=w261:string)  [unwired: 14 in]
      }
      frame "UI: Update When Start" {
        w264 = cluster{"f0":dbl, "df":dbl, "magnitude":dbl[]}[] [] ("FFT")
        # "Enable: Stop\nDisable: Start, Exit, Settings"
        n98 = property on="AnalysisWnd 1" class="WFGraph (strict)"("Value"=w264) -> ()  [unwired: 2 in, 2 out]
        n99 = property on="AnalysisWnd 2" class="WFGraph (strict)"("Value"=w264) -> ()  [unwired: 2 in, 2 out]
        n100 = property on="WaveformGraph" class="WFChart (strict)"("History Data"=waveform(dbl)[][] []) -> ()  [unwired: 2 in, 2 out]
        n101 = Unbundle By Name(w266) -> ("UI Refs.Stop Ref"=w272:refnum<vi>, "UI Refs.Start Ref"=w271:refnum<vi>, "UI Refs.Exit Ref"=w270:refnum<vi>, "UI Refs.Settings Ref"=w269:refnum<vi>, "UI Refs.Data Source Ref"=w265:refnum<vi>)
        n102 = Build Array(w271, w270, w269, w265) -> (w274:refnum<vi>[])
        n103 = Build Array(w272) -> (w273:refnum<vi>[])
        n104 = call "Set Enable State on Multiple Controls.vi"("Enable?"=TRUE, "Controls"=w273) -> ()  [unwired: 10 in]
        n105 = call "Set Enable State on Multiple Controls.vi"("Enable?"=FALSE, "Controls"=w274) -> ()  [unwired: 10 in]
      }
      frame "UI: Update When Stop" {
        # "Enable: Start, Exit, Settings\nDisable: Stop"
        n106 = Unbundle By Name(w279) -> ("UI Refs.Stop Ref"=w284:refnum<vi>, "UI Refs.Start Ref"=w285:refnum<vi>, "UI Refs.Exit Ref"=w286:refnum<vi>, "UI Refs.Settings Ref"=w287:refnum<vi>, "UI Refs.Data Source Ref"=w278:refnum<vi>)
        n107 = Build Array(w285, w286, w287, w278) -> (w282:refnum<vi>[])
        n108 = Build Array(w284) -> (w283:refnum<vi>[])
        n109 = call "Set Enable State on Multiple Controls.vi"("Enable?"=FALSE, "Controls"=w283) -> ()  [unwired: 10 in]
        n110 = call "Set Enable State on Multiple Controls.vi"("Enable?"=TRUE, "Controls"=w282) -> ()  [unwired: 10 in]
      }
      frame "UI: Cursor Set" {
        # "Argument"
        # "Set and Unset Cursor Busy.\n(Usage: \"UI: Cursor Set >> Busy|Idle\")"
        n111 = disable-structure shown="Default" {
          disable-tunnel: w294 -> [w300 w305]
          disable-tunnel: [w299 w305] -> w293
          disable-tunnel: w292 -> [w298 _]
          frame condition #0 (active) {
            n112 = case shown="\"Busy\"" w298 {
              tunnel: w300 -> [w302 w304]
              tunnel: [w301 w303] -> w299
              frame "Idle", Default {
                n113 = call <vilib>:"Unset Busy.vi"("error in (no error)"=w302) -> ("error out"=w301:errorcluster)  [unwired: 10 in]
              }
              frame "Busy" {
                n114 = call <vilib>:"Set Busy.vi"("error in (no error)"=w304) -> ("error out"=w303:errorcluster)  [unwired: 9 in, 1 out]
              }
            }
          }
          frame condition #1 {
          }
        }
        n115 = call <vilib>:"Add State(s) to Queue__JKI_lib_State_Machine.vi"("State(s) in (\"\")"=w297) -> ("States Out"=w296:string)  [unwired: 14 in]
      }
      frame "UI: Front Panel State" {
        # "Argument"
        # "Set Front Panel Open or Closed\n(Usage: \"UI: Front Panel State >> Open|Close\")"
        n116 = Unbundle By Name(w309) -> ("Core.Current VI Reference"=w308:refnum<vi>)
        n117 = case shown="\"Minimize\", \"Minimized\"" w307 {
          tunnel: w311 -> [w319 w334 w345 w358 w371]
          tunnel: [w321 w335 w347 w360 w373] -> w310
          tunnel: w308 -> [w320 w332 w346 w359 w372]
          frame "Open", "Standard", Default {
            w314 = T3."Standard" ("State")
            n118 = property class="VI"(reference=w320, error in=w319) -> (reference out=w317:refnum<vi>, error out=w318:errorcluster, "FP.State"=w316:T3)
            n119 = Not Equal?(x=w316, y=w314) -> (x != y?=w315:bool)
            n120 = case shown="True" w315 {
              tunnel: [w325 w327] -> w321
              tunnel: w318 -> [w324 w327]
              tunnel: w317 -> [w323 _]
              tunnel: w314 -> [w322 _]
              frame True {
                n121 = invoke class="VI" method="FP.Open"(reference=w323, error in=w324, "Activate"=TRUE, "State"=w322) -> (error out=w325:errorcluster)  [unwired: 1 in, 4 out]
              }
              frame False {
              }
            }
          }
          frame "Close", "Closed" {
            n122 = property class="VI"(reference=w332, error in=w334) -> (reference out=w331:refnum<vi>, error out=w333:errorcluster, "FP.State"=w329:T3)
            n123 = Not Equal?(x=w329, y=T3."Closed" ("Front Panel Window:State")) -> (x != y?=w328:bool)
            n124 = case shown="True" w328 {
              tunnel: [w336 w339] -> w335
              tunnel: w333 -> [w336 w338]
              tunnel: w331 -> [_ w337]
              frame False {
              }
              frame True {
                n125 = invoke class="VI" method="FP.Close"(reference=w337, error in=w338) -> (error out=w339:errorcluster)  [unwired: 1 in, 2 out]
              }
            }
          }
          frame "Hidden", "Hide" {
            w340 = T3."Hidden" ("State")
            n126 = property class="VI"(reference=w346, error in=w345) -> (reference out=w343:refnum<vi>, error out=w344:errorcluster, "FP.State"=w342:T3)
            n127 = Not Equal?(x=w342, y=w340) -> (x != y?=w341:bool)
            n128 = case shown="True" w341 {
              tunnel: [w351 w352] -> w347
              tunnel: w344 -> [w350 w352]
              tunnel: w343 -> [w349 _]
              tunnel: w340 -> [w348 _]
              frame True {
                n129 = invoke class="VI" method="FP.Open"(reference=w349, error in=w350, "State"=w348) -> (error out=w351:errorcluster)  [unwired: 2 in, 4 out]
              }
              frame False {
              }
            }
          }
          frame "Minimize", "Minimized" {
            w353 = T3."Minimized" ("State")
            n130 = property class="VI"(reference=w359, error in=w358) -> (reference out=w356:refnum<vi>, error out=w357:errorcluster, "FP.State"=w355:T3)
            n131 = Not Equal?(x=w355, y=w353) -> (x != y?=w354:bool)
            n132 = case shown="True" w354 {
              tunnel: [w364 w365] -> w360
              tunnel: w357 -> [w363 w365]
              tunnel: w356 -> [w362 _]
              tunnel: w353 -> [w361 _]
              frame True {
                n133 = invoke class="VI" method="FP.Open"(reference=w362, error in=w363, "State"=w361) -> (error out=w364:errorcluster)  [unwired: 2 in, 4 out]
              }
              frame False {
              }
            }
          }
          frame "Maximize", "Maximized" {
            w366 = T3."Maximized" ("State")
            n134 = property class="VI"(reference=w372, error in=w371) -> (reference out=w369:refnum<vi>, error out=w370:errorcluster, "FP.State"=w368:T3)
            n135 = Not Equal?(x=w368, y=w366) -> (x != y?=w367:bool)
            n136 = case shown="True" w367 {
              tunnel: [w377 w378] -> w373
              tunnel: w370 -> [w376 w378]
              tunnel: w369 -> [w375 _]
              tunnel: w366 -> [w374 _]
              frame True {
                n137 = invoke class="VI" method="FP.Open"(reference=w375, error in=w376, "State"=w374) -> (error out=w377:errorcluster)  [unwired: 2 in, 4 out]
              }
              frame False {
              }
            }
          }
        }
        n138 = call <vilib>:"Add State(s) to Queue__JKI_lib_State_Machine.vi"("State(s) in (\"\")"=w313) -> ("States Out"=w312:string)  [unwired: 14 in]
      }
      frame "UI: Change Waveform Graph Legend Num" {
        n139 = Unbundle By Name(w385) -> ("UI Refs.Data Ref"=w384:refnum<vi>)
        n140 = call "Convert API String Arguments to Data.vim"("Reference Type"=u32 0 ("Legend:Number of Rows"), "API String"=w382) -> ("error out"=w380:errorcluster, "Data"=w383:u32)  [unwired: 6 in]
        n141 = property class="WFChart (strict)"(reference=w384, error in=w380, "LegNumRows"=w383) -> (error out=w379:errorcluster)  [unwired: 1 out]
      }
      frame "UI: Update Waveform Graph" {
        n142 = call "CSM - Convert Argument to MassData.vim"("Type"=waveform(dbl)[] [] ("Data"), "MassData Argument"=w400) -> ("error out"=w398:errorcluster, "Data"=w394:waveform(dbl)[])  [unwired: 6 in]
        "WaveformGraph" <- w394
        n143 = Array Size(array=w394) -> (size(s)=w391:i32)
        n144 = feedback-in #1(w391) -> ()
        n145 = feedback #1(0) -> (w392:i32)
        n146 = Not Equal?(x=w391, y=w392) -> (x != y?=w388:bool)
        n147 = Format Into String(w391) -> (resulting string=w393:string)  [unwired: 3 in, 1 out]
        n148 = call <vilib>:"Build State String with Arguments__JKI_lib_State_Machine.vi"("Arguments (\"\")"=w393, "State"="UI: Change Waveform Graph Legend Num") -> ("State with Arguments"=w389:string)  [unwired: 4 in]
        n149 = call-poly <userlib>:"Add State(s) to Queue By BOOL++.vi"("TRUE (\"\")"=w389, "Condition"=w388, "State Queue (\"\")"=w396) -> ("Remaining States"=w397:string)  [unwired: 8 in]
      }
      frame "UI: Update AnalysisWnd 1" {
        n150 = call "CSM - Convert Argument to MassData.vim"("Type"=cluster{"f0":dbl, "df":dbl, "magnitude":dbl[]}[] [] ("FFT - (RMS)"), "MassData Argument"=w406) -> ("error out"=w405:errorcluster, "Data"=→"AnalysisWnd 1":cluster{"f0":dbl, "df":dbl, "magnitude":dbl[]}[])  [unwired: 6 in]
      }
      frame "UI: Update AnalysisWnd 2" {
        n151 = call "CSM - Convert Argument to MassData.vim"("Type"=cluster{"f0":dbl, "df":dbl, "magnitude":dbl[]}[] [] ("FFT - (RMS)"), "MassData Argument"=w413) -> ("error out"=w412:errorcluster, "Data"=→"AnalysisWnd 2":cluster{"f0":dbl, "df":dbl, "magnitude":dbl[]}[])  [unwired: 6 in]
      }
      frame "---------- Macro ----------" {
        n152 = call <vilib>:"Add State(s) to Queue__JKI_lib_State_Machine.vi"("State(s) in (\"\")"=w421) -> ("States Out"=w420:string)  [unwired: 14 in]
      }
      frame "Macro: Initialize" {
        w422 = "Data: Initialize\nInitialize Core Data\nEvents: Register\nUI: Initialize\nUI: Front Panel State >> Open\nUI: Change Waveform Graph Legend Num >> 1\nDO: Update Status >> Ready...\n\n//Permanent registrations\nAcquired Waveform@Acquisition >> API: Log@Logging -><register>\nAcquired Waveform@Acquisition >> UI: Update Waveform Graph -><register>\n\n//Dynamic registrations\nMacro: Register Analysis Relationships"  # Data: Initialize Initialize Core Data Events: Register UI: Initialize UI: Front Panel State >> Open UI: Change Waveform Graph Legend Num >> 1 DO: Update Status >> Ready...  //Permanent registrations Acquired Waveform@Acquisition >> API: Log@Logging -><register> Acquired Waveform@Acquisition >> UI: Update Waveform Graph -><register>  //Dynamic registrations Macro: Register Analysis Relationships
        # "Initialization Macro\n(This is called once, when the VI starts)"
        n153 = call <userlib>:"CSM - Populate Configuration Variables.vi"("String with INI-Variable"=w422) -> ("String"=w423:string)  [unwired: 7 in, 1 out]
        n154 = call <vilib>:"Add State(s) to Queue__JKI_lib_State_Machine.vi"("State(s) in Front (\"\")"=w423, "State(s) in (\"\")"=w428) -> ("States Out"=w427:string)  [unwired: 13 in]
      }
      frame "Macro: Register Analysis Relationships" {
        # "<2>"
        # "<1>"
        # "#CSM-NOTE\n<1> and <2> will be replaced."
        # "#CSM-NOTE\nState could be registered as status. It's similar to Status with response as its argument."
        n155 = Format Into String("Analysis Window 1") -> (resulting string=w430:string)  [unwired: 3 in, 1 out]
        n156 = Format Into String("Analysis Window 2") -> (resulting string=w429:string)  [unwired: 3 in, 1 out]
        n157 = call-poly <userlib>:"Build Message with Arguments++.vi"("States With Replace Token"="//Dynamic registrations\n\n//For AnalysisWnd 1\nAcquired Waveform@Acquisition >> API: <1>@Algorithm -><register>\nAPI: <1>@Algorithm >> UI: Update AnalysisWnd 1 -><register>\n//For AnalysisWnd 2\nAcquired Waveform@Acquisition >> API: <2>@Algorithm -><register>\nAPI: <2>@Algorithm >> UI: Update AnalysisWnd 2 -><register>" ("State(s) in Front (\"\")"), "<1>"=w430, "<2>"=w429) -> ("States"=w433:string)  [unwired: 12 in]
        n158 = Bundle By Name(cluster=w439, "Relationships"=w433) -> (w435:T9)
        n159 = call <vilib>:"Add State(s) to Queue__JKI_lib_State_Machine.vi"("State(s) in Front (\"\")"=w433, "State(s) in (\"\")"=w436) -> ("States Out"=w437:string)  [unwired: 13 in]
      }
      frame "Macro: Unregister Analysis Relationships" {
        n160 = Unbundle By Name(w451) -> ("Relationships"=w450:string)
        n161 = Search and Replace String(replace all?=TRUE ("ignore case? (F)"), case sensitive?=TRUE ("ignore case? (F)"), input string=w450, search string="<register>" ("replace string (\"\")"), replace string="<unregister>" ("replace string (\"\")")) -> (result string=w443:string)  [unwired: 3 in, 3 out]
        n162 = Bundle By Name(cluster=w451, "Relationships"="") -> (w442:T9)
        n163 = call <vilib>:"Add State(s) to Queue__JKI_lib_State_Machine.vi"("State(s) in Front (\"\")"=w443, "State(s) in (\"\")"=w444) -> ("States Out"=w445:string)  [unwired: 13 in]
      }
      frame "Macro: Start" {
        n164 = Bundle By Name(cluster=w458, "State"=UI_State."Acquiring and Logging" ("UI State")) -> (w457:T9)
        n165 = call <vilib>:"Add State(s) to Queue__JKI_lib_State_Machine.vi"("State(s) in Front (\"\")"="//Local States\nDO: Update Status >> Acquiring and Logging...\nUI: Update When Start\n\n//Send Message to Other CSM Modules\nAPI: Start -@ Logging\nAPI: Start ->| Acquisition" ("State(s) in Front (\"\")"), "State(s) in (\"\")"=w455) -> ("States Out"=w456:string)  [unwired: 13 in]
      }
      frame "Macro: Stop" {
        n166 = Unbundle By Name(w462) -> ("State"=w464:T5)
        n167 = case shown="Default" w464 {
          selector: w464 -> [w471 _]
          tunnel: [w471 UI_State."Waiting for Stop" ("UI State")] -> w463
          frame "Waiting for Exit" {
          }
          frame Default {
          }
        }
        n168 = Bundle By Name(cluster=w462, "State"=w463) -> (w468:T9)
        n169 = call <vilib>:"Add State(s) to Queue__JKI_lib_State_Machine.vi"("State(s) in Front (\"\")"="//Local States\nDO: Update Status >> Stopping...\nUI: Update When Stop\n\n//Send Message to Other CSM Modules\nAPI: Stop -@ Acquisition\nAPI: Stop -@ Logging\n" ("State(s) in Front (\"\")"), "State(s) in (\"\")"=w466) -> ("States Out"=w467:string)  [unwired: 13 in]
      }
      frame "Macro: Exit" {
        w480 = "//UI: Front Panel State >> Close"  # //UI: Front Panel State >> Close
        w477 = "//Dynamic registrations\nMacro: Unregister Analysis Relationships\n\n//Permanent registrations\nAcquired Waveform@Acquisition >> API: Log@Logging -><unregister>\nAcquired Waveform@Acquisition >> UI: Update Waveform Graph -><unregister>\n\nData: Cleanup\nEvents: Unregister\nExit"  # //Dynamic registrations Macro: Unregister Analysis Relationships  //Permanent registrations Acquired Waveform@Acquisition >> API: Log@Logging -><unregister> Acquired Waveform@Acquisition >> UI: Update Waveform Graph -><unregister>  Data: Cleanup Events: Unregister Exit
        # "Exit Macro\n(This is called once, when the VI exits)"
        n170 = Unbundle By Name(w482) -> ("Core.Close Panel on Exit?"=w481:bool)
        n171 = disable-structure shown="Enabled" {
          disable-tunnel: [w485 w497 w503] -> w474
          disable-tunnel: w473 -> [_ w496 _]
          frame Disabled {
            w492 = "Macro: Exit -@ Acquisition\nMacro: Exit -@ Logging"  # Macro: Exit -@ Acquisition Macro: Exit -@ Logging
            n172 = call <userlib>:"CSM - Module Status.vi"("CSM Name"="Algorithm") -> ("#Nodes"=w488:i32, "CSM Name (Dup)"=w490:string)  [unwired: 6 in, 3 out]
            n173 = for {
              N: w488 -> [_]
              tunnel: w490 -> [w495]
              tunnel: "Macro: Exit" -> [w494]
              tunnel: [w493] -> w486 mode=indexing
              n174 = call-poly <userlib>:"Build Message with Arguments++.vi"("State With Arguments"=w494, "Target Module (\"\")"=w495) -> ("CSM Message String"=w493:string)  [unwired: 13 in]
            }
            n175 = Build Array (concatenate)(w492, w486) -> (w487:string[])
            n176 = call <userlib>:"CSM - Compact Multiple States.vi"("Multiple States"=w487) -> ("States"=w485:string)  [unwired: 9 in]
          }
          frame Enabled {
            # "#NOTE\nHelper VI is equivalent to other case"
            n177 = call <userlib>:"CSM - List Modules.vi"() -> ("Module Names"=w499:string[])  [unwired: 10 in, 1 out]
            n178 = Search 1D Array(1D array=w499, element=w496) -> (index of element=w500:i32)  [unwired: 1 in]
            n179 = Delete From Array(array=w499, index=w500) -> (array with subset deleted=w498:string[])  [unwired: 1 in, 1 out]
            n180 = call <userlib>:"CSM - Build Exit Messages of CSMs.vi"("State With Arguments (\"Macro: Exit“)"="Macro: Exit" ("State with Arguments(\"Macro: Exit“)"), "CSMs"=w498) -> ("States"=w497:string)  [unwired: 13 in]
          }
          frame Disabled {
            # "#NOTE\nHelper VI is equivalent to other case"
            n181 = call <userlib>:"CSM - Build Exit Messages of CSMs.vi"("State With Arguments (\"Macro: Exit“)"="Macro: Exit" ("State with Arguments(\"Macro: Exit“)"), "CSMs"=string[] ["Acquisition", "Logging", "Algorithm"]) -> ("States"=w503:string)  [unwired: 13 in]
          }
        }
        n182 = Select(t=w480, s=w481, f="") -> (s? t:f=w478:string)
        n183 = call <vilib>:"Add State(s) to Queue__JKI_lib_State_Machine.vi"("State(s) in Front (\"\")"=w474, "State(s) in (\"\")"=w478, "State(s) at Back (\"\")"=w477) -> ("States Out"=w476:string)  [unwired: 12 in]
        n184 = call <vilib>:"Add State(s) to Queue__JKI_lib_State_Machine.vi"("State(s) in Front (\"\")"=w476, "State(s) in (\"\")"=w484) -> ("States Out"=w483:string)  [unwired: 13 in]
      }
      frame "---------- DoSth ----------" {
        n185 = call <vilib>:"Add State(s) to Queue__JKI_lib_State_Machine.vi"("State(s) in (\"\")"=w509) -> ("States Out"=w508:string)  [unwired: 14 in]
      }
      frame "Do: Update Status" {
        n186 = call <vilib>:"Add State(s) to Queue__JKI_lib_State_Machine.vi"("State(s) in (\"\")"=w515) -> ("States Out"=w514:string)  [unwired: 14 in]
        "Status" <- w510
      }
      frame "Do: Launch Settings Dialog" {
        # "Your code here.\n(You can make a copy of, or modify, this frame)"
        n187 = call <userlib>:"CSM - Check If Module Exists.vi"("CSM Name"="Acquisition" ("Name(\"\" to use uuid)")) -> ("error out"=w522:errorcluster, "Exist?"=w518:bool, "CSM Name (Dup)"=w520:string)  [unwired: 8 in]
        n188 = case shown="True" w518 {
          tunnel: w522 -> [w530 w542]
          tunnel: w520 -> [w526 w541]
          tunnel: w519 -> [_ w540]
          tunnel: [w529 w539] -> w517
          frame False {
            n189 = Format Into String(format string="Cannot Find the CSM which named %s !!!", w526) -> (resulting string=w525:string)  [unwired: 2 in, 1 out]
            n190 = Bundle By Name(cluster=w530, "status"=TRUE, "source"=w525) -> (w529:errorcluster)
          }
          frame True {
            w534 = T3."Standard" ("State")
            n191 = call <userlib>:"CSM - Module VI Reference.vi"("Current Module (\"\" to Generate an ID)"=w540, "error in (no error)"=w542, "Force? (F)"=TRUE ("force?(F)"), "CSM Name"=w541) -> ("error out"=w532:errorcluster, "CSM Module VIRef"=w533:refnum<vi>)  [unwired: 6 in]
            n192 = property class="VI"(reference=w533, error in=w532) -> (reference out=w537:refnum<vi>, error out=w538:errorcluster, "FP.State"=w536:T3)
            n193 = Not Equal?(x=w536, y=w534) -> (x != y?=w535:bool)
            n194 = case shown="True" w535 {
              tunnel: [w549 w551] -> w539
              tunnel: w538 -> [w544 w551]
              tunnel: w537 -> [w543 _]
              tunnel: w534 -> [w548 _]
              frame True {
                n195 = property class="VI"(reference=w543, error in=w544, "FP.Behavior"=T6."Modal" ("Front Panel Window:Behavior")) -> (reference out=w546:refnum<vi>, error out=w547:errorcluster)
                n196 = invoke class="VI" method="FP.Open"(reference=w546, error in=w547, "Activate"=TRUE, "State"=w548) -> (error out=w549:errorcluster)  [unwired: 1 in, 4 out]
              }
              frame False {
              }
            }
          }
        }
      }
      frame "Do: Confirm Quit" {
        n197 = Unbundle By Name(w556) -> ("State"=w559:T5)
        n198 = case shown="\"Acquiring and Logging\"" w559 {
          tunnel: [UI_State."Idle" ("UI State") w568] -> w558
          tunnel: w556 -> [w563 w567]
          tunnel: [w563 w566] -> w557
          tunnel: [TRUE w565] -> w552
          frame Default {
          }
          frame "Acquiring and Logging" {
            n199 = Two Button Dialog(message="Are you sure you want to quit while the acquisition is running?" ("Confirm Quit Message"), 1:"No" ("No"), 2:"Yes" ("Yes")) -> (T button?=w569:bool)
            n200 = case shown="False" w569 {
              tunnel: [UI_State."Acquiring and Logging" ("UI State") UI_State."Waiting for Exit" ("UI State")] -> w568
              tunnel: w567 -> [w573 w576]
              tunnel: [w573 w576] -> w566
              tunnel: [_ TRUE] -> w565
              frame False {
                # "User did not want to quit."
              }
              frame True {
              }
            }
          }
        }
        n201 = Bundle By Name(cluster=w557, "State"=w558) -> (w555:T9)
        n202 = call-poly <userlib>:"Add State(s) to Queue By BOOL++.vi"("TRUE (\"\")"="Macro: Exit", "Condition"=w552, "State Queue (\"\")"=w561) -> ("Remaining States"=w554:string)  [unwired: 8 in]
      }
    }
  }
  n203 = call <userlib>:"CSM - Sync Configuration Variables to File.vi"("All Temp Variable to Default Ini(F)"=TRUE, "error in (no error)"=w2) -> ("error out"=w1:errorcluster)  [unwired: 7 in]
  n204 = disable-structure shown="RUN_TIME_ENGINE==True" {
    disable-tunnel: w1 -> [_ _]
    frame condition #0 (active) {
    }
    frame condition #1 {
      n205 = Quit LabVIEW(quit? (T)=TRUE) -> ()
    }
  }
